vi "Set Tag.vi"(8 "error in (no error)":errorcluster, 10 "Tag":string, 11 "CTI_GPIO_DigitalOut in":refnum<class "CTI_GPIO_DigitalOut.lvclass">) -> (0 "error out":errorcluster, 3 "CTI_GPIO_DigitalOut out":refnum<class "CTI_GPIO_DigitalOut.lvclass">)   [LabVIEW 2021, in "CTI_GPIO_DigitalOut.lvclass"]
uses:
  CTI_GPIO_DigitalOut.lvclass
  CTI_GPIO_DigitalOut.lvclass/CTI_GPIO_DigitalOut.ctl
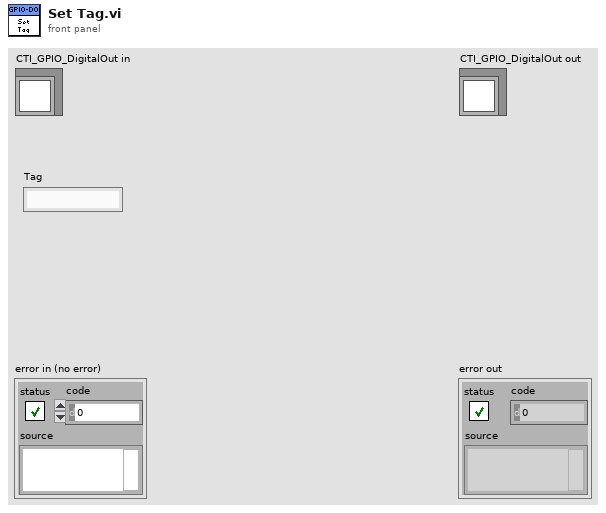
[diagram p1: front panel]
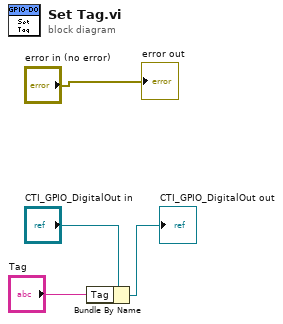
[diagram p0: block diagram]
diagram:
  n1 = Bundle By Name(cluster="CTI_GPIO_DigitalOut in", "Tag"="Tag") -> (→"CTI_GPIO_DigitalOut out":refnum<class "CTI_GPIO_DigitalOut.lvclass">)
  "error out" <- "error in (no error)"
